vi "Settling_V_to_Pa.vi"(0 "sens_mV_per_psi":dbl=1.26, 1 "Actual_AI_Rate":dbl=300300.3, 2 "V_array":dbl[](array[numeric]), 3 "gain":dbl=1.0, 4 "baseline_ms":dbl=10.0) -> (5 "P_Pa_array":dbl[](array[numeric]))   [LabVIEW 2025]
uses:
  <vilib>/Analysis/baseanly.llb/Mean (DBL).vi
  <vilib>/Analysis/NI_AALBase.lvlib
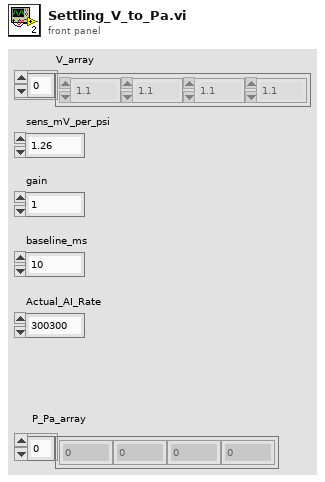
[diagram p1: front panel]
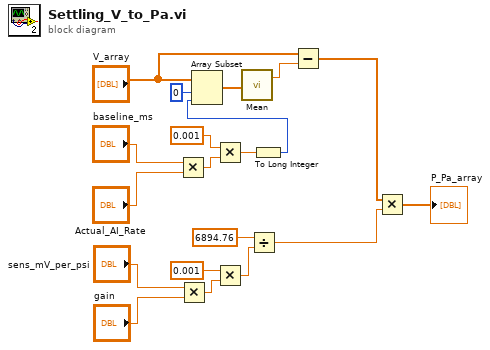
[diagram p0: block diagram]
diagram:
  n1 = Multiply(x="baseline_ms", y="Actual_AI_Rate") -> (x*y=w17:dbl)
  n2 = Multiply(x="sens_mV_per_psi", y="gain") -> (x*y=w8:dbl)
  n3 = Multiply(x=0.001, y=w17) -> (x*y=w2:dbl)
  n4 = Multiply(x=0.001, y=w8) -> (x*y=w6:dbl)
  n5 = Divide(x=6894.76, y=w6) -> (x/y=w4:dbl)
  n6 = To Long Integer(number=w2) -> (32bit integer=w1:i32)
  n7 = Array Subset(array="V_array", index=0, length=w1) -> (w15:dbl[])
  n8 = call-poly <vilib>:"Mean.vi"("X"=w15) -> ("mean"=w12:dbl)  [unwired: 1 out]
  n9 = Subtract(x="V_array", y=w12) -> (x-y=w5:dbl[])
  n10 = Multiply(x=w5, y=w4) -> (x*y=→"P_Pa_array":dbl[])
